vi "Scale Values.vi"(8 "error in (no error)":errorcluster, 10 "Values":dbl[](array[numeric]), 11 "VolatusScaling in":refnum<class "Scaling.lvclass">) -> (0 "error out":errorcluster, 2 "Scaled Values":dbl[](array[numeric]), 3 "VolatusScaling out":refnum<class "Scaling.lvclass">)   [LabVIEW 2020, in "VolatusData.lvlib" / "Scaling.lvclass"]
uses:
  Scaling.lvclass
  Scaling.lvclass/Scaling.ctl
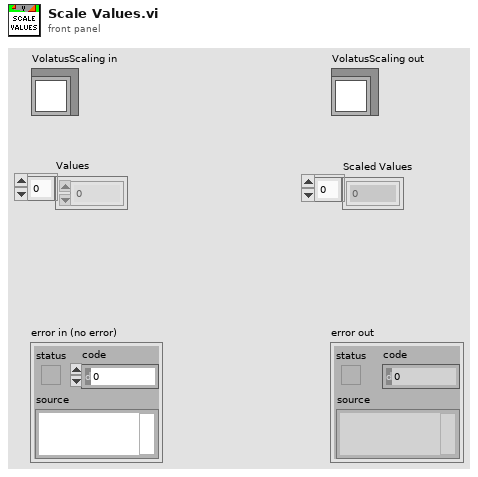
[diagram p1: front panel]
types:
  T1 = typedef "VolatusConfig.lvlib/Scale Type.ctl" = enum16{"None", "Sensor", "Polynomial", "Threshold", "Invert Bool"}
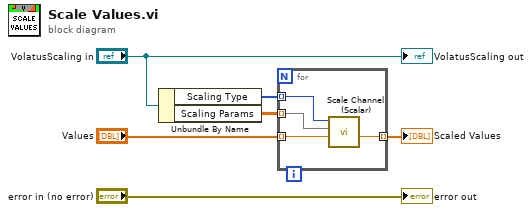
[diagram p0: block diagram]
diagram:
  n1 = Unbundle By Name("VolatusScaling in") -> ("Scaling Type"=w2:T1[], "Scaling Params"=w3:dbl[][])
  n2 = for {
    tunnel: "Values" -> [w10] mode=indexing
    tunnel: w3 -> [w8] mode=indexing
    tunnel: w2 -> [w7] mode=indexing
    tunnel: [w9] -> w1 mode=indexing
    n3 = call "Scale Channel (Scalar).vi"("Value"=w10, "Scaling Params"=w8, "Scaling Type"=w7) -> ("Scaled Value"=w9:dbl)  [unwired: 8 in]
  }
  "Scaled Values" <- w1
  "error out" <- "error in (no error)"
  "VolatusScaling out" <- "VolatusScaling in"
